vi "04-nested_data_structures.vi"() -> ()   [LabVIEW 2018, in "LV2Julia_examples.lvlib"]
uses:
  LV2Julia_examples.lvlib
  LV2Julia_core/VIs/Server or client state.ctl
  LV2Julia_core/VIs/detailed error info.ctl
  LV2Julia_core/VIs/StackFrame.ctl
  LV2Julia_core/VIs/Commands.ctl
  8e064ee8-a8f1-4e0c-9ba7-d24acaf12b18.vi
  c1a008e0-c205-4ae9-8ab0-5de19ea2baa8.vi
  f6dd2d06-6566-45f8-9309-3186a7d78478.vi
  <vilib>/Utility/High Resolution Relative Seconds.vi
  c1a008e0-c205-4ae9-8ab0-5de19ea2baa8.vi/1e4f0138-484c-4844-8f87-c91e2f5cc599.vi
  c1a008e0-c205-4ae9-8ab0-5de19ea2baa8.vi/1e4f0138-484c-4844-8f87-c91e2f5cc599.vi/54deefdc-66bd-4efb-b043-23a1ea9a35e0.vi
  c1a008e0-c205-4ae9-8ab0-5de19ea2baa8.vi/1e4f0138-484c-4844-8f87-c91e2f5cc599.vi/124a22fe-574f-4dba-bb8a-7905f090a076.vi
  c1a008e0-c205-4ae9-8ab0-5de19ea2baa8.vi/1e4f0138-484c-4844-8f87-c91e2f5cc599.vi/2cfaf326-5419-4260-b137-2c8c0cda3a8c.vi
  LV2Julia_core/VIs/jl-scripts path.vi
  LV2Julia_core/VIs/check ID validity.vi
  LV2Julia_core/VIs/bindata_descr to JSON.vi
  LV2Julia_core/VIs/check cluster field names.vi
  LV2Julia_core/VIs/concat JSON.vi
  LV2Julia_core/VIs/build request.vi
  LV2Julia_core/VIs/Parse server response.vi
  LV2Julia_core/VIs/log jl exceptions.vi
  LV2Julia_core/LV2Julia_core.lvlib
panel:
  out "call duration (ms)":dbl format="%#.2f"
  out "returned value":T1
  in  "Argument":T2={"text_data"="eh?", "num_data"={"factor"=2, "num_arr"=[3.14, 2.72, 1.62]}} {"num_data"."num_arr" format="%#.2f"}
  in  "next":bool
  out "detailed error info":T3
  out "current error":errorcluster
  out "final error":errorcluster
  out "short err code":u8
  in  "stop":bool
  out "ZMQ timeout":bool
  out "Julia script file path":path
  out "temporary script path":path
  out "Jl Server state":T5
  # "Here the same (nested) data structure for the argument and returned value: for simplicity only."
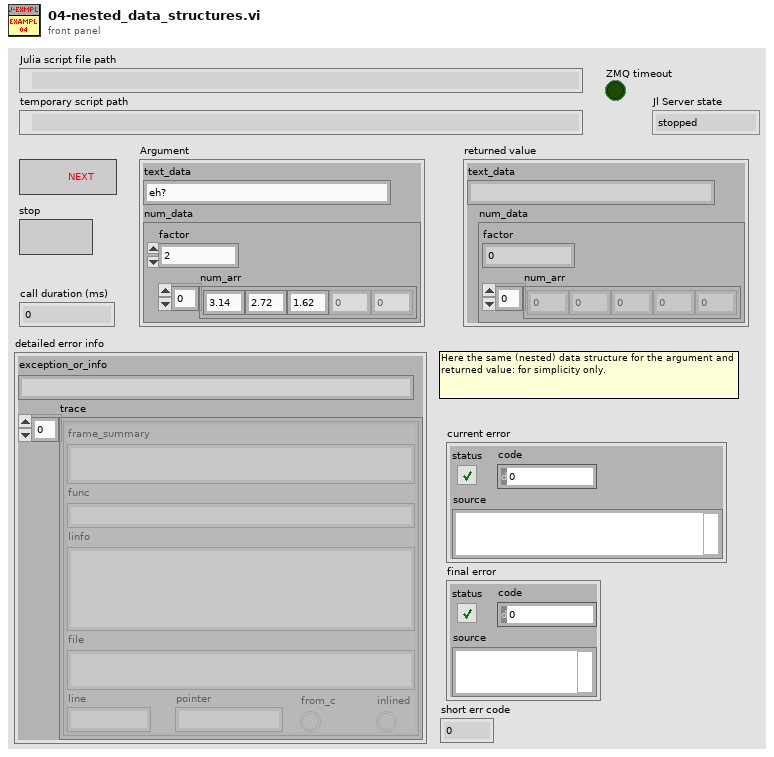
[diagram p1: front panel]
types:
  T1 = cluster{"text_data":string, "num_data":cluster{"factor":i32, "num_arr":dbl[]}}
  T2 = cluster{"text_data":string, "num_data":cluster{"factor":u64, "num_arr":dbl[]}}
  T3 = typedef "LV2Julia_core.lvlib/detailed error info.ctl" = cluster{"exception_or_info":string, "trace":T4[]}
  T4 = typedef "LV2Julia_core.lvlib/StackFrame.ctl" = cluster{"frame_summary":string, "func":string, "linfo":string, "file":string, "line":i32, "pointer":u64, "from_c":bool, "inlined":bool}
  T5 = typedef "LV2Julia_core.lvlib/Server or client state.ctl" = enum16{"stopped", "running", "unknown"}
  T6 = typedef "LV2Julia_core.lvlib/Commands.ctl" = enum16{"Start Jl-server & Init LV-client", "Send request & Get response ", "Stop Jl-server & Cleanup LV-client", "Cleanup LV-client", "Start Jl-server", "Stop Jl-server", "Init LV-Client", "Cleanup LV-Client", "(not allowed)", "Set LV Client state", "Set Jl Server state", "set ZMQ timeout", "read ZMQ timeout", "read-out state"}
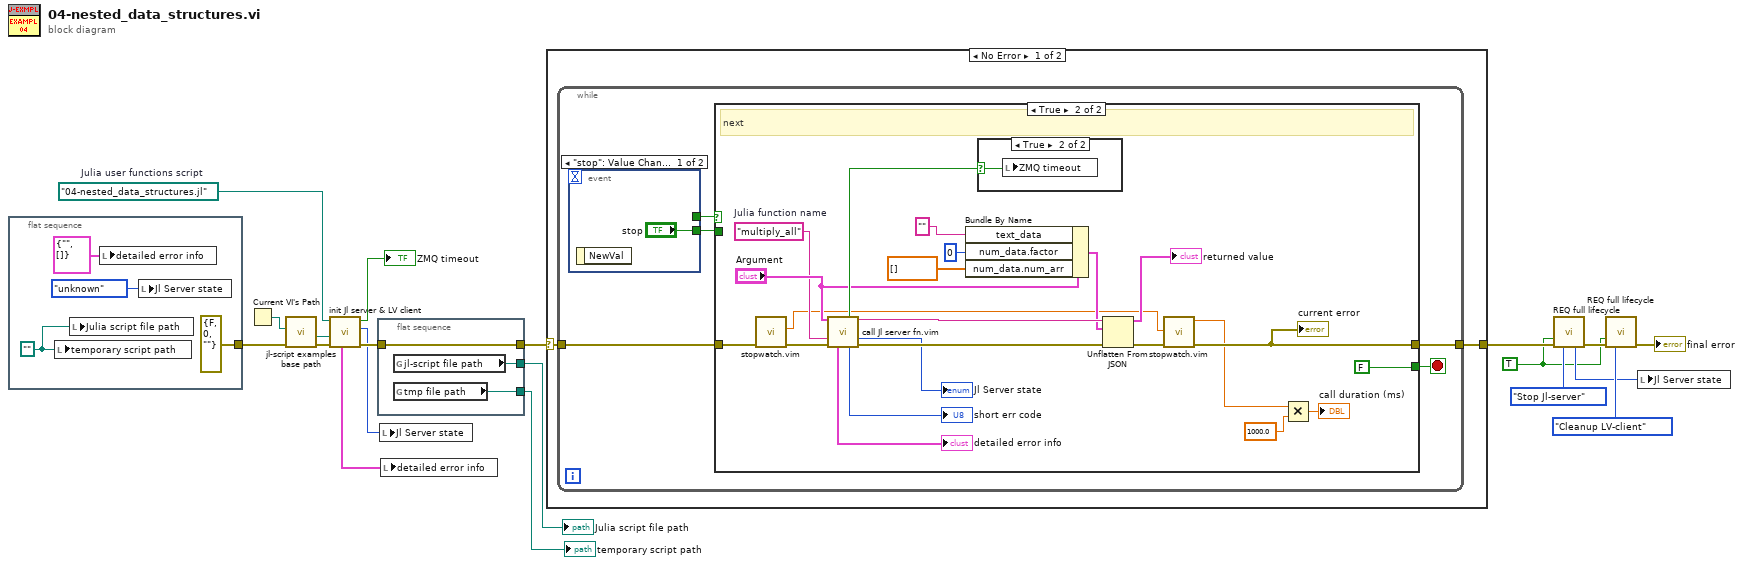
[diagram p0: block diagram]
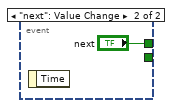
[diagram p2: hidden frame]
diagram:
  w6 = path "04-nested_data_structures.jl"  # Julia user functions script
  w10 = TRUE ("Force command")
  n1 = flat-sequence {
    tunnel: [errorcluster {"status"=FALSE, "code"=0, "source"=""} ("error in (no error)")] -> w2
    frame #0 {
      w20 = path ""
      n2 = local write "temporary script path"(w20) -> ()
      n3 = local write "Julia script file path"(w20) -> ()
      n4 = local write "detailed error info"(T3 {"exception_or_info"="", "trace"=[]} ("detailed error info")) -> ()
      n5 = local write "Jl Server state"(Server_or_client_state."unknown" ("Jl Server state out")) -> ()
    }
  }
  n6 = Current VI's Path() -> (path=w5:path)
  n7 = call "jl-script examples base path.vi"("error in (no error)"=w2, "calling example VI path"=w5) -> ("error out"=w4:errorcluster, "jl-script-examples base path"=w3:path)  [unwired: 8 in]
  n8 = call "init Jl server & LV client.vi"("error in (no error)"=w4, "Base path (not a path)"=w3, "Julia user functions script"=w6) -> ("error out"=w9:errorcluster, "Jl Server state out"=w7:T5, "timeout?"=→"ZMQ timeout":bool, "detailed error info"=w1:T3)  [unwired: 3 in, 2 out]
  n9 = flat-sequence {
    tunnel: [w26] -> w14
    tunnel: w9 -> [w26]
    tunnel: [w25] -> w12
    tunnel: [w24] -> w13
    frame #0 {
      n10 = global read "jl-scripts path.vi" "jl-script file path"() -> (w25:path)
      n11 = global read "jl-scripts path.vi" "tmp file path"() -> (w24:path)
    }
  }
  n12 = local write "Jl Server state"(w7) -> ()
  n13 = local write "detailed error info"(w1) -> ()
  n14 = case shown="No Error" w14 {
    selector: w14 -> [w27 w61]
    tunnel: [w28 w61] -> w19
    frame No Error {
      n15 = while {
        tunnel: w27 -> [w32]
        tunnel: [w33] -> w28
        stop <- w30 stop-if-true
        n16 = event shown="[0] \"stop\": Value Change" {
          selector: _ -> [_ _]
          dyn-events: _ -> [_ _]
          timeout: _ -> [_ _]
          tunnel: [_ "next"] -> w31
          tunnel: ["stop" _] -> w29
          event "stop": Value Change {
            n17 = event-data() -> ()  [unwired: 1 in, 1 out]
          }
          event "next": Value Change {
            n18 = event-data() -> ()  [unwired: 1 in, 1 out]
          }
        }
        n19 = case shown="True" w31 {
          tunnel: [w37 w39] -> w33
          tunnel: w32 -> [w37 w43]
          tunnel: [w36 FALSE ("stop this VI only")] -> w30
          tunnel: w29 -> [w36 _]
          frame False {
            # "stop"
          }
          frame True {
            w51 = "multiply_all"  # Julia function name
            # "next"
            n20 = call "stopwatch.vim"("anything in"=w43) -> ("copy of anything out"=w42:errorcluster, "current timepoint"=w40:dbl)  [unwired: 8 in, 1 out]
            n21 = call "call Jl server fn.vim"("Arguments 1"="Argument", "fun2call"=w51, "error in (no error)"=w42) -> ("timeout?"=w53:bool, "JSON received"=w50:string, "Jl Server state out"=→"Jl Server state":T5, "detailed error info"=→"detailed error info":T3, "return code"=→"short err code":u8, "error out"=w57:errorcluster)  [unwired: 6 in, 1 out]
            n22 = Bundle By Name(cluster="Argument", "text_data"="", "num_data.factor"=u32 0, "num_data.num_arr"=dbl[] []) -> (w47:T2)
            n23 = case shown="True" w53 {
              selector: w53 -> [_ w60]
              frame False {
              }
              frame True {
                n24 = local write "ZMQ timeout"(w60) -> ()
              }
            }
            n25 = Unflatten From JSON(JSON string=w50, type and defaults=w47, error in (no error)=w57) -> (value=→"returned value":T2, error out=w41:errorcluster)  [unwired: 4 in]
            n26 = call "stopwatch.vim"("anything in"=w41, "prev timepoint (0)"=w40) -> ("copy of anything out"=w39:errorcluster, "delta t (s)"=w38:dbl)  [unwired: 7 in, 1 out]
            "current error" <- w39
            n27 = Multiply(x=w38, y=1000.0) -> (x*y=→"call duration (ms)":dbl)
          }
        }
      }
    }
    frame Error {
    }
  }
  n28 = call "REQ full lifecycle.vi"("Force command"=w10, "error in"=w19, "command"=Commands."Stop Jl-server") -> ("Jl Server state out"=w11:T5, "error out"=w17:errorcluster)  [unwired: 6 in, 5 out]
  n29 = call "REQ full lifecycle.vi"("Force command"=w10, "error in"=w17, "command"=Commands."Cleanup LV-client") -> ("error out"=→"final error":errorcluster)  [unwired: 6 in, 6 out]
  n30 = local write "Jl Server state"(w11) -> ()
  "temporary script path" <- w13
  "Julia script file path" <- w12
